vi "SPARK Configure Absolute Encoder.vi"   [LabVIEW 2023]
doc: "Configure an absolute encoder connected to the data port of the SPARK."
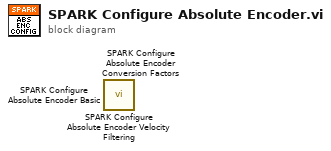
[diagram p0: block diagram]
diagram:
  n1 = call <vilib>:"SPARK Configure Absolute Encoder Velocity Filtering.vi"() -> ()  [unwired: 10 in, 2 out]
  n2 = call <vilib>:"SPARK Configure Absolute Encoder Conversion Factors.vi"() -> ()  [unwired: 10 in, 2 out]
  n3 = call <vilib>:"SPARK Configure Absolute Encoder Basic.vi"() -> ()  [unwired: 10 in, 2 out]
